vi "HTTP Client reqwest Tree.vi"() -> ()   [LabVIEW 2020]
uses:
  <vilib>/VIPM Community/HTTP Client Plugin - Base/Classes/Abstract HTTP Client/Abstract HTTP Client.lvclass
  HTTP Client reqwest.lvclass
  usr/local/natinst/LabVIEW-2024-64/vi.lib/VIPM Community/HTTP Client Plugin - Base/Classes/Abstract HTTP Client/Abstract HTTP Client.lvclass
  <vilib>/Utility/error.llb/DialogType.ctl
panel:
  out "status code":u32[](array[numeric])
  in  "timeout (10000)":i32=10000
  out "Array":string[][](array[string])
  # "reqwest"
  # "built-in"
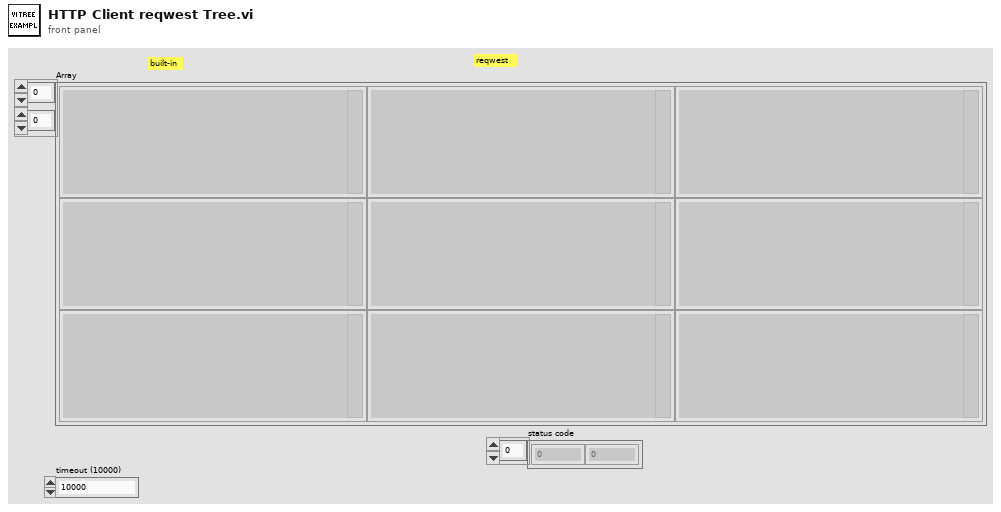
[diagram p1: front panel]
types:
  T1 = typedef "DialogType.ctl" = u16
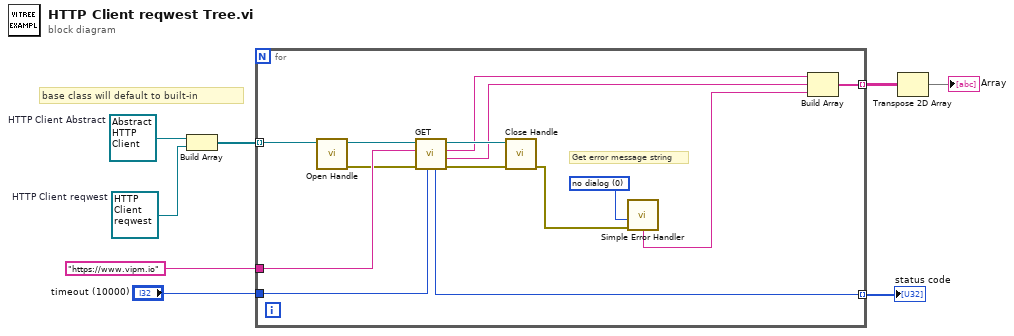
[diagram p0: block diagram]
diagram:
  w3 = refnum<class "HTTP Client reqwest.lvclass"> refnum  # HTTP Client reqwest
  w4 = refnum<class "Abstract HTTP Client.lvclass"> refnum  # HTTP Client Abstract
  # "base class will default to built-in"
  n1 = Build Array(w4, w3) -> (w8:refnum<class "Abstract HTTP Client.lvclass">[])
  n2 = for {
    tunnel: w8 -> [w22] mode=indexing
    tunnel: "https://www.vipm.io" ("url") -> [w19]
    tunnel: [w15] -> w6 mode=indexing
    tunnel: "timeout (10000)" -> [w13]
    tunnel: [w12] -> w1 mode=indexing
    w9 = T1 0 items=["no dialog", "OK message", "continue or stop message", "OK message + warnings", "continue/stop + warnings"] ("type of dialog (OK msg:1)")
    # "Get error message string"
    n3 = call-dynamic "Open Handle.vi"("HTTP Client Abstract in"=w22) -> ("error out"=w18:errorcluster, "HTTP Client Abstract out"=w21:refnum<class "Abstract HTTP Client.lvclass">)  [unwired: 9 in]
    n4 = call-dynamic "GET.vi"("timeout (10000)"=w13, "error in (no error)"=w18, "url"=w19, "HTTP Client Abstract in"=w21) -> ("error out"=w17:errorcluster, "body"=w14:string, "headers"=w16:string, "HTTP Client Abstract out"=w20:refnum<class "Abstract HTTP Client.lvclass">, "status code"=w12:u32)  [unwired: 3 in]
    n5 = call-dynamic "Close Handle.vi"("error in (no error)"=w17, "HTTP Client Abstract in"=w20) -> ("error out"=w11:errorcluster)  [unwired: 8 in, 1 out]
    n6 = call <vilib>:"Simple Error Handler.vi"("type of dialog (OK msg:1)"=w9, "error in (no error)"=w11) -> ("message"=w10:string)  [unwired: 3 in, 4 out]
    n7 = Build Array(w16, w14, w10) -> (w15:string[])
  }
  "status code" <- w1
  n8 = Transpose 2D Array(2D array=w6) -> (transposed array=→"Array":string[][])
